vi "TCP call.vi"(7 "port":u16=5000, 9 "data string in":string, 10 "JSON string in":string) -> (1 "data string out":string, 2 "JSON string out":string)   [LabVIEW 2020, in "LabVIEW-Python TCP Lib.lvlib"]
uses:
  LabVIEW-Python TCP Lib.lvlib
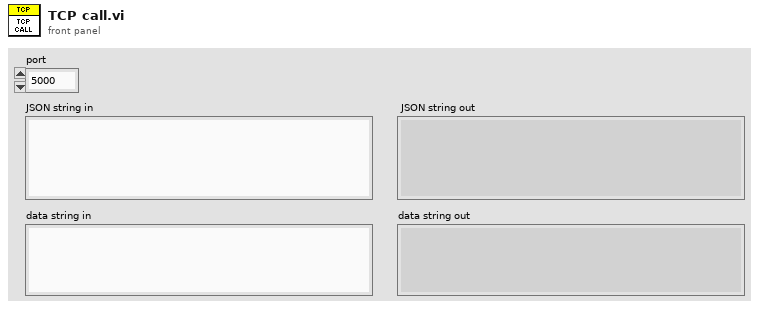
[diagram p1: front panel]
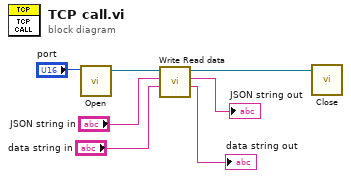
[diagram p0: block diagram]
diagram:
  n1 = call "Open.vi"("port"="port") -> ("connection ID"=w6:refnum<k5>)  [unwired: 9 in, 1 out]
  n2 = call "Write Read data.vi"("data string in"="data string in", "JSON string in"="JSON string in", "connection ID"=w6) -> ("data string out"=→"data string out":string, "JSON string out"=→"JSON string out":string, "connection ID out"=w2:refnum<k5>)  [unwired: 5 in, 1 out]
  n3 = call "Close.vi"("connection ID"=w2) -> ()  [unwired: 9 in, 2 out]
